vi "test 9401 DIO FPGA Mode Loop Back.vi"(8 "error in (no error)":errorcluster, 11 "TestCase in":refnum<class "Scan Engine EtherCAT System Tests.lvclass">) -> (0 "error out":errorcluster, 3 "TestCase out":refnum<class "Scan Engine EtherCAT System Tests.lvclass">)   [LabVIEW 2020, in "Scan Engine EtherCAT System Tests.lvclass"]
uses:
  Scan Engine EtherCAT System Tests.lvclass
  C:/Program Files (x86)/National Instruments/LabVIEW 2020/vi.lib/NI/VeriStand Custom Device Testing Tools/VeriStandTestCase/VeriStandTestCase.lvclass
  <vilib>/addons/_JKI Toolkits/VI Tester/TestCase.llb/TestCase.lvclass
  <vilib>/NI/VeriStand Custom Device Testing Tools/VeriStandTestCase/VeriStandTestCase.lvclass
  System Explorer/SEECD System Explorer.lvlib
  C:/Program Files (x86)/National Instruments/LabVIEW 2020/vi.lib/addons/_JKI Toolkits/VI Tester/TestCase.llb/TestCase.lvclass
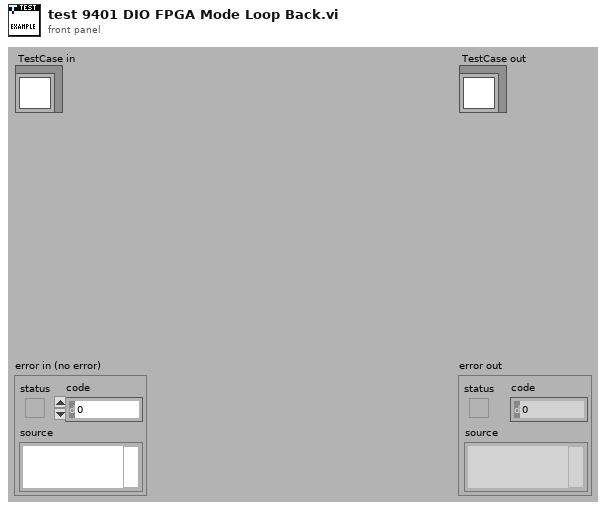
[diagram p1: front panel]
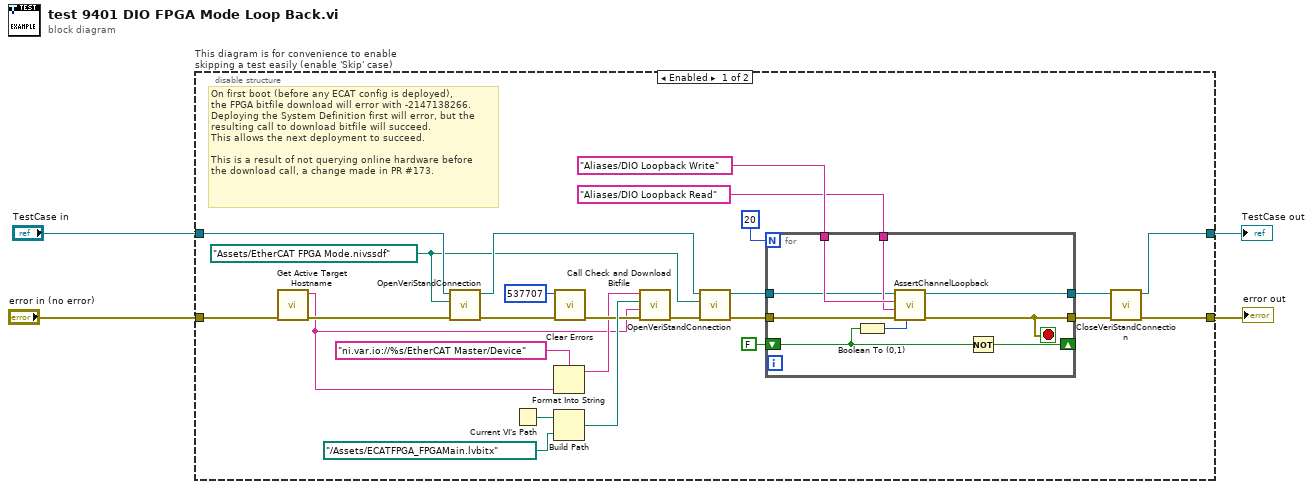
[diagram p0: block diagram]
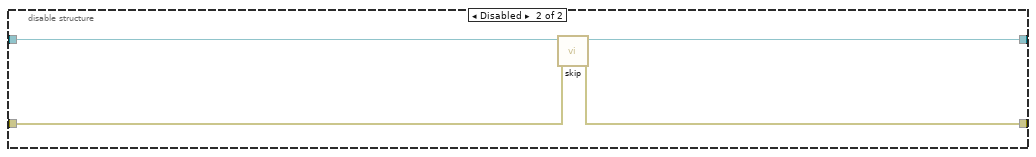
[diagram p2: hidden frame]
diagram:
  n1 = disable-structure "This diagram is for convenience to enable skipping a test easily (enable 'Skip' case)" shown="Enabled" {
    disable-tunnel: "TestCase in" -> [w12 w42]
    disable-tunnel: [w20 w40] -> w1
    disable-tunnel: [w21 w41] -> w3
    disable-tunnel: "error in (no error)" -> [w9 w39]
    frame Enabled {
      w11 = path "Assets/EtherCAT FPGA Mode.nivssdf" ("System Definition File")
      # "On first boot (before any ECAT config is deployed),\nthe FPGA bitfile download will error with -2147138266.\nDeploying the System Definition first will error, but the\nresulting call to download bitfile will succeed.\nThis allows the next deployment to succeed.\n\nThis is a result of not querying online hardware before\nthe download call, a change made in PR #173."
      n2 = call "Get Active Target Hostname.vi"("error in"=w9) -> ("error out"=w8:errorcluster, "IP Address / Hostname"=w5:string)  [unwired: 9 in]
      n3 = call-dynamic "OpenVeriStandConnection.vi"("error in (no error)"=w8, "System Definition File"=w11, "VeriStand Test Case in"=w12) -> ("error out"=w14:errorcluster, "VeriStand Test Case out"=w13:refnum<class "Scan Engine EtherCAT System Tests.lvclass">)  [unwired: 6 in, 1 out]
      n4 = Current VI's Path() -> (path=w17:path)
      n5 = Format Into String(format string="ni.var.io://%s/EtherCAT Master/Device", w5) -> (resulting string=w6:string)  [unwired: 2 in, 1 out]
      n6 = Build Path(base path=w17, name or relative path=path "../Assets/ECATFPGA_FPGAMain.lvbitx" ("bitfile path in")) -> (appended path=w16:path)
      n7 = call <vilib>:"Clear Errors.vi"("error in (no error)"=w14, "specific error code to clear (0: all)"=537707) -> ("error out"=w15:errorcluster)  [unwired: 4 in, 1 out]
      n8 = call "Call Check and Download Bitfile.vi"("error in"=w15, "Target IP Address"=w5, "Bitfile Path"=w16, "Slave Ref"=w6) -> ("error out"=w19:errorcluster)  [unwired: 7 in]
      n9 = call-dynamic "OpenVeriStandConnection.vi"("error in (no error)"=w19, "System Definition File"=w11, "VeriStand Test Case in"=w13) -> ("error out"=w25:errorcluster, "VeriStand Test Case out"=w24:refnum<class "Scan Engine EtherCAT System Tests.lvclass">)  [unwired: 6 in, 1 out]
      n10 = for {
        N: 20 -> [_]
        tunnel: "Aliases/DIO Loopback Write" ("Channel") -> [w35]
        tunnel: [w33] -> w23
        tunnel: "Aliases/DIO Loopback Read" ("Channel") -> [w34]
        shift-right: [w38] -> _
        shift-left: FALSE -> [w37]
        tunnel: w25 -> [w36]
        tunnel: [w30] -> w22
        tunnel: w24 -> [w31]
        stop <- w33 stop-if-true
        n11 = Boolean To (0,1)(Boolean=w37) -> (0, 1=w32:i16)
        n12 = call <vilib>:"AssertChannelLoopback.vi"("Value"=w32, "error in (no error)"=w36, "Read Channel"=w34, "Write Channel"=w35, "VeriStand Test Case in"=w31) -> ("error out"=w33:errorcluster, "VeriStand Test Case out"=w30:refnum<class "Scan Engine EtherCAT System Tests.lvclass">)  [unwired: 5 in]
        n13 = Not(x=w37) -> (.not. x?=w38:bool)
      }
      n14 = call-dynamic "CloseVeriStandConnection.vi"("error in (no error)"=w23, "VeriStand Test Case in"=w22) -> ("error out"=w21:errorcluster, "VeriStand Test Case out"=w20:refnum<class "Scan Engine EtherCAT System Tests.lvclass">)  [unwired: 8 in]
    }
    frame Disabled {
      n15 = call <vilib>:"skip.vi"("error in (no error)"=w39, "TestCase in"=w42) -> ("error out"=w41:errorcluster, "TestCase out"=w40:refnum<class "Scan Engine EtherCAT System Tests.lvclass">)  [unwired: 8 in]
    }
  }
  "error out" <- w3
  "TestCase out" <- w1
